vi "Destroy.vi"(8 "error in (no error)":errorcluster, 11 "CIF_Iceoryx_BB in":refnum<class "CIF_Iceoryx_BB.lvclass">) -> (0 "error out":errorcluster, 3 "CIF_Iceoryx_BB out":refnum<class "CIF_Iceoryx_BB.lvclass">)   [LabVIEW 2021, in "CIF_Iceoryx_BB.lvclass"]
uses:
  CIF_Iceoryx_BB.lvclass
  CIF_Iceoryx_BB.lvclass/CIF_Iceoryx_BB.ctl
  ChannelCommon/typedef/Channel State.ctl
  ChannelCommon/ChannelCommon.lvlib
  3af3f266-2185-4c49-8968-ef3a3bbd4b7e.vi
  <vilib>/CIF Foundation/CIF Iceoryx/Refnum/Typedef/BB Reader Refnum.ctl
  <vilib>/CIF Foundation/CIF Iceoryx/Iceoryx.lvlib
  Typedef/Data Configuration.ctl
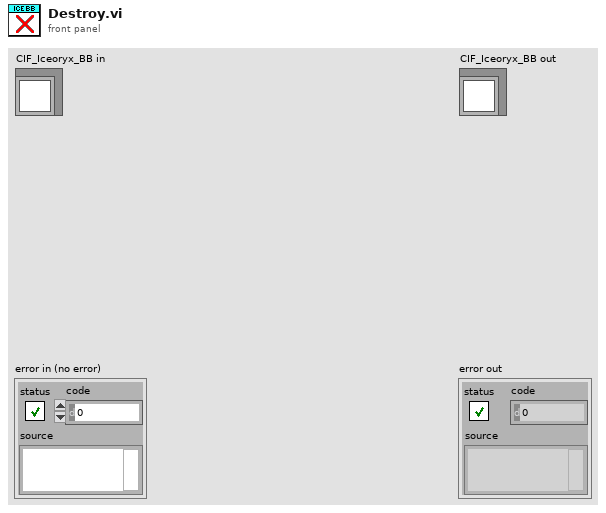
[diagram p1: front panel]
types:
  T1 = typedef "CIF_Iceoryx_BB.lvclass/Data Configuration.ctl" = cluster{"Element Size":u32, "Element Alignment":u32, "Array":bool, "Type":string}
  T2 = typedef "Iceoryx.lvlib/BB Reader Refnum.ctl" = cluster{"refnum":u64, "BB Reader":enum8{"bb_reader"}}
  T3 = typedef "ChannelCommon.lvlib/Channel State.ctl" = enum8{"Creating", "Disconnected", "Connecting", "Connected", "Destroyed"}
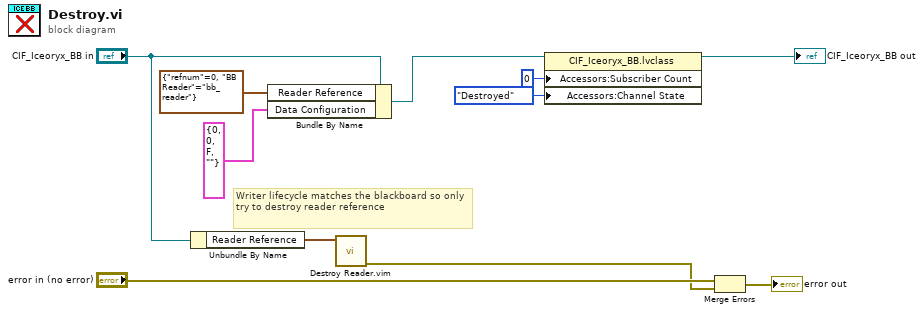
[diagram p0: block diagram]
diagram:
  # "Writer lifecycle matches the blackboard so only try to destroy reader reference"
  n1 = Unbundle By Name("CIF_Iceoryx_BB in") -> ("Reader Reference"=w6:T2)
  n2 = Bundle By Name(cluster="CIF_Iceoryx_BB in", "Reader Reference"=T2 {"refnum"=0, "BB Reader"=enum."bb_reader"}, "Data Configuration"=T1 {"Element Size"=0, "Element Alignment"=0, "Array"=FALSE, "Type"=""}) -> (w1:refnum<class "CIF_Iceoryx_BB.lvclass">)
  n3 = call "Destroy Reader.vim"("Reader Reference"=w6) -> ("error out"=w5:errorcluster)  [unwired: 10 in]
  n4 = property class="CIF_Iceoryx_BB.lvclass"(reference=w1, "Accessors:Subscriber Count"=u32 0 ("Subscriber Count"), "Accessors:Channel State"=Channel_State."Destroyed" ("Channel State")) -> (reference out=→"CIF_Iceoryx_BB out":refnum<class "CIF_Iceoryx_BB.lvclass">)  [unwired: 1 in, 1 out]
  n5 = Merge Errors("error in (no error)", w5) -> (→"error out":errorcluster)
